vi "IV2-LCRZ.vi"(0 "Voltage In":cdb=-0.04516796338063459+0.012130821220646867i format="%#_4p", 1 "Test Frequency":dbl=25000.0, 5 "Current In":cdb=0.0013952524174977166+0.030636391761552667i format="%#_4p", 12 "LCR Params":T2={"Rg_Vmon"=5000.0, "Rg_Imon"=5000.0, "ESL_Cal"=2.95e-07, "ESR_Cal"=0.0, "Cp_Cal"=0.0, "Rp_Cal"=1000000000.0, "Use Open/Short\nCompensation"=TRUE, "R_Shunt"=100.0, "RLoad"=1000000000.0, "RLoad_Meas"=1000000000.0} {"RLoad_Meas" format="%#_6p"; "RLoad" format="%#_6p"}) -> (4 "Impedance (Mag)":dbl=0.0009831918388061723 format="%#_3p", 6 "Impedance (Phase)":dbl=169.4760326381836 format="%#_3p", 8 "Ls":dbl=9.665874386883538e-10 format="%#_3p", 10 "Cs":dbl=-0.029973703968004497 format="%#_3p", 14 "Impedance cluster":T3={"|Z|"=0.0009831918388061723, "Phase(Z)"=169.4760326381836, "Re(Z)"=-0.000966653166475792, "Imag(Z)"=0.00017957685718763175, "Ls"=9.665874386883538e-10, "Cs"=-0.029973703968004497, "Rp"=0.0, "Cp"=0.0}, 15 "Real (Z)":dbl=-0.000966653166475792 format="%#_3p")   [LabVIEW 2021]
panel:
  out "Z":cdb
  out "Y":cdb
  in  "Cal Cluster":T1={"ESL_Cal"=2e-07, "ESR_Cal"=0.0, "Cp_Cal"=0.0, "Rp_Cal"=1000000000.0, "RLoad"=1000000000.0, "RLoad_Meas"=1000000000.0} {"RLoad_Meas" format="%#_6p"; "RLoad" format="%#_6p"}
  out "Current Phase\nDeg":dbl=87.39241896335173
  out "Z Phase (Pre)":dbl=77.5743267290552
  out "Z Mag (pre-correction)":dbl=152.4989366461181
  out "VGain":dbl=11.0 format="%#_3p"
  out "Detected Current\n(Measured Signal \nmagnitude)":dbl=0.030668146821675832 format="%#_3p"
  out "I_Gain":dbl=11.0 format="%#_3p"
  out "Imag(Z)":dbl=0.00017957685718763175 format="%#_3p"
  out "Voltage (mag)":dbl=0.004251690708375082 format="%#_3p"
  out "Current  (Amps)":dbl=2.7880133474250757e-05 format="%#_3p"
  out "Voltage Phase\n (deg)":dbl=164.96674569240693 format="%.2p"
  out "Detected Voltage\n(Measured Signal\nMagnitude":dbl=0.0467685977921259 format="%.2p"
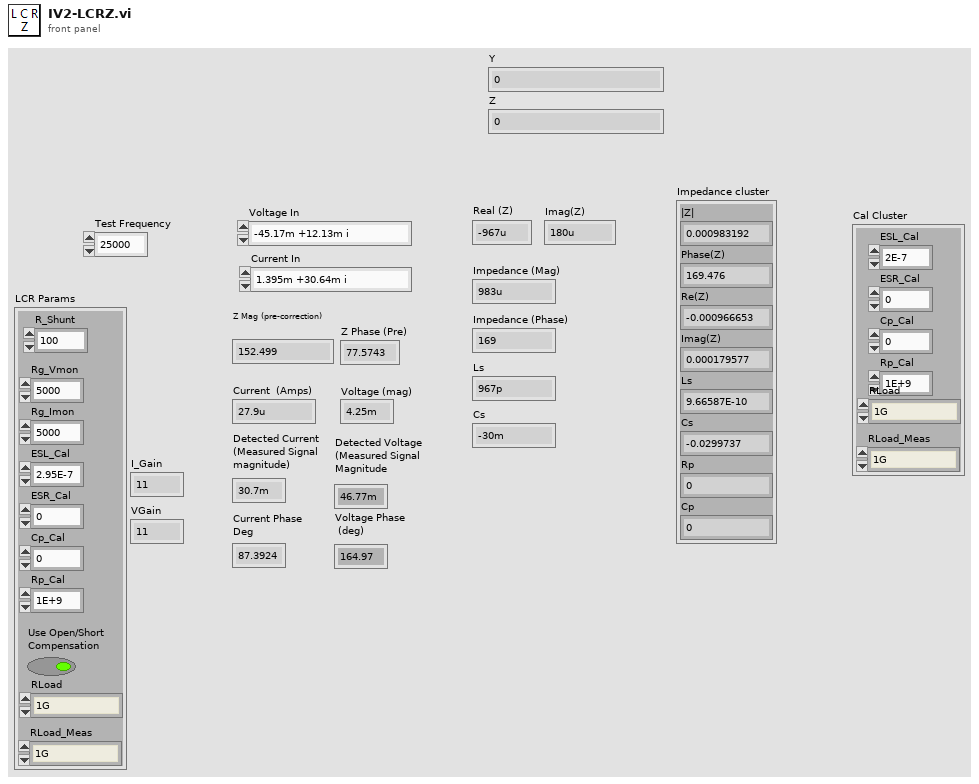
[diagram p1: front panel]
types:
  T1 = cluster{"ESL_Cal":dbl, "ESR_Cal":dbl, "Cp_Cal":dbl, "Rp_Cal":dbl, "RLoad":dbl, "RLoad_Meas":dbl}
  T2 = cluster{"Rg_Vmon":dbl, "Rg_Imon":dbl, "ESL_Cal":dbl, "ESR_Cal":dbl, "Cp_Cal":dbl, "Rp_Cal":dbl, "Use Open/Short\nCompensation":bool, "R_Shunt":dbl, "RLoad":dbl, "RLoad_Meas":dbl}
  T3 = cluster{"|Z|":dbl, "Phase(Z)":dbl, "Re(Z)":dbl, "Imag(Z)":dbl, "Ls":dbl, "Cs":dbl, "Rp":dbl, "Cp":dbl}
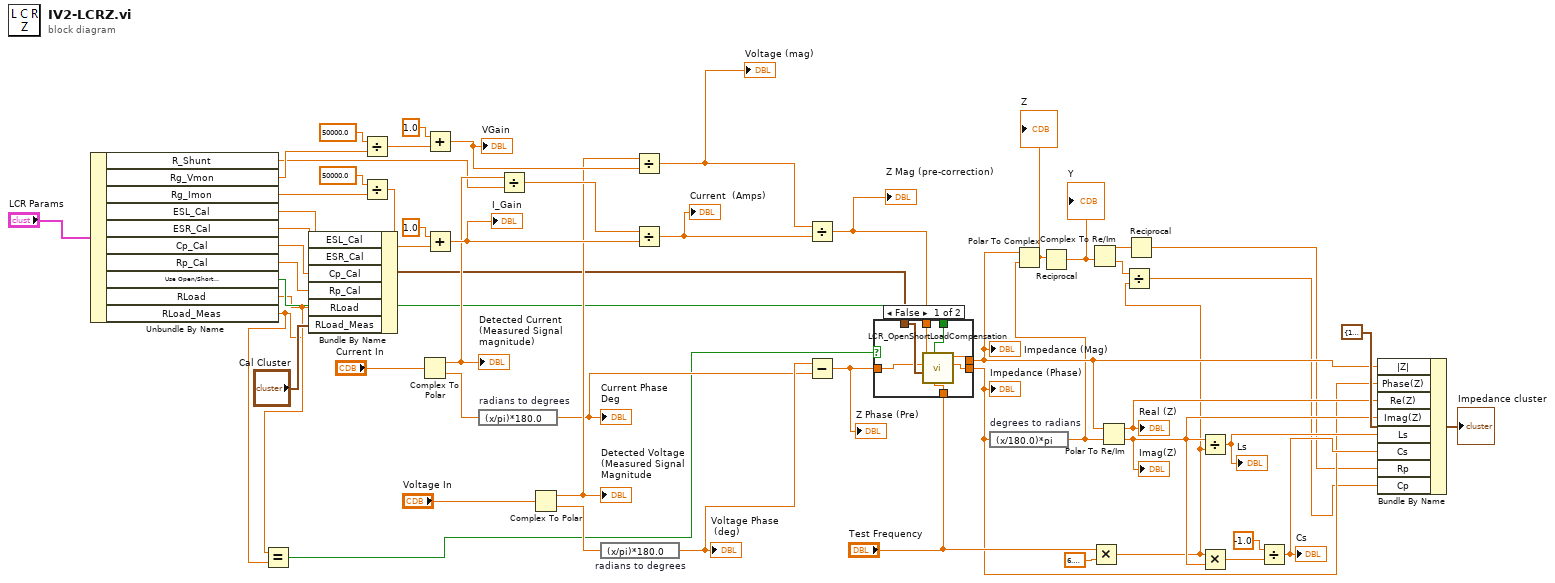
[diagram p0: block diagram]
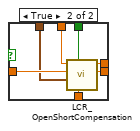
[diagram p2: hidden frame]
diagram:
  n1 = Unbundle By Name("LCR Params") -> ("R_Shunt"=w15:dbl, "Rg_Vmon"=w17:dbl, "Rg_Imon"=w18:dbl, "ESL_Cal"=w22:dbl, "ESR_Cal"=w21:dbl, "Cp_Cal"=w20:dbl, "Rp_Cal"=w19:dbl, "Use Open/Short\nCompensation"=w16:bool, "RLoad"=w2:dbl, "RLoad_Meas"=w1:dbl)
  n2 = Equal?(x=w2, y=w1) -> (x = y?=w3:bool)
  n3 = Bundle By Name(cluster="Cal Cluster", "ESL_Cal"=w22, "ESR_Cal"=w21, "Cp_Cal"=w20, "Rp_Cal"=w19, "RLoad"=w2, "RLoad_Meas"=w1) -> (w14:T1)
  n4 = Divide(x=50000.0, y=w17) -> (x/y=w47:dbl)
  n5 = Divide(x=50000.0, y=w18) -> (x/y=w51:dbl)
  n6 = Complex To Polar(r * e^(i*theta)="Current In") -> (r=w39:dbl, theta=w34:dbl)
  "Detected Current\n(Measured Signal \nmagnitude)" <- w39
  n7 = Add(x=1.0, y=w47) -> (x+y=w44:dbl)
  "VGain" <- w44
  n8 = Add(x=1.0, y=w51) -> (x+y=w49:dbl)
  "I_Gain" <- w49
  n9 = expression code="(x/pi)*180.0" "radians to degrees"(w34) -> (w33:dbl)
  "Current Phase\nDeg" <- w33
  n10 = Divide(x=w39, y=w15) -> (x/y=w50:dbl)
  n11 = Complex To Polar(r * e^(i*theta)="Voltage In") -> (r=w40:dbl, theta=w36:dbl)
  "Detected Voltage\n(Measured Signal\nMagnitude" <- w40
  n12 = expression code="(x/pi)*180.0" "radians to degrees"(w36) -> (w35:dbl)
  "Voltage Phase\n (deg)" <- w35
  n13 = Divide(x=w40, y=w44) -> (x/y=w43:dbl)
  "Voltage (mag)" <- w43
  n14 = Divide(x=w50, y=w49) -> (x/y=w48:dbl)
  "Current  (Amps)" <- w48
  n15 = Divide(x=w43, y=w48) -> (x/y=w41:dbl)
  "Z Mag (pre-correction)" <- w41
  n16 = Subtract(x=w35, y=w33) -> (x-y=w42:dbl)
  "Z Phase (Pre)" <- w42
  n17 = case shown="False" w3 {
    tunnel: w42 -> [w58 w69]
    tunnel: w41 -> [w57 w68]
    tunnel: "Test Frequency" -> [w60 w67]
    tunnel: w16 -> [w56 w66]
    tunnel: w14 -> [w59 w65]
    tunnel: [w62 w64] -> w13
    tunnel: [w61 w63] -> w12
    frame False {
      n18 = call "LCR_OpenShortLoadCompensation.vi"("Freq"=w60, "UseCorrection"=w56, "Cal Cluster"=w59, "Phase Z Meas Deg"=w58, "Mag Z Meas"=w57) -> ("Phase Z DUT"=w61:dbl, "Mag Z DUT"=w62:dbl)  [unwired: 4 in, 1 out]
    }
    frame True {
      n19 = call "LCR_OpenShortCompensation.vi"("Freq"=w67, "UseCorrection"=w66, "Cal Cluster"=w65, "Phase Z Meas Deg"=w69, "Mag Z Meas"=w68) -> ("Phase Z DUT"=w63:dbl, "Mag Z DUT"=w64:dbl)  [unwired: 4 in, 1 out]
    }
  }
  "Impedance (Mag)" <- w13
  "Impedance (Phase)" <- w12
  n20 = expression code="(x/180.0)*pi" "degrees to radians"(w12) -> (w4:dbl)
  n21 = Polar To Complex(1:w4, 2:w13) -> (0:w11:cdb)
  "Z" <- w11
  n22 = Reciprocal(x=w11) -> (1/x=w10:cdb)
  "Y" <- w10
  n23 = Complex To Re/Im(x + iy=w10) -> (x=w9:dbl, y=w7:dbl)
  n24 = Multiply(x="Test Frequency", y=6.283185307179586) -> (x*y=w6:dbl)
  n25 = Polar To Re/Im(2:w4, 3:w13) -> (0:w28:dbl, 1:w29:dbl)
  "Imag(Z)" <- w28
  "Real (Z)" <- w29
  n26 = Divide(x=w7, y=w6) -> (x/y=w5:dbl)
  n27 = Reciprocal(x=w9) -> (1/x=w8:dbl)
  n28 = Divide(x=w28, y=w6) -> (x/y=w27:dbl)
  "Ls" <- w27
  n29 = Multiply(x=w6, y=w28) -> (x*y=w55:dbl)
  n30 = Divide(x=-1.0, y=w55) -> (x/y=w26:dbl)
  "Cs" <- w26
  n31 = Bundle By Name(cluster=T3 {"|Z|"=1.0, "Phase(Z)"=0.0, "Re(Z)"=1.0, "Imag(Z)"=0.0, "Ls"=1.0, "Cs"=1.0, "Rp"=1.0, "Cp"=1.0}, "|Z|"=w13, "Phase(Z)"=w12, "Re(Z)"=w29, "Imag(Z)"=w28, "Ls"=w27, "Cs"=w26, "Rp"=w8, "Cp"=w5) -> (→"Impedance cluster":T3)
